vi "Create filename.vi"(9 "Number":i32, 10 "Parameters":T1={"Time"=0.0, "Pixels X"=1, "Pixels Y"=1, "Max galvo"=0.0, "Min galvo"=0.0} {"Pixels Y" min=1; "Pixels X" min=1 step=1; "Time" min=1.0}, 11 "Comment":string) -> (3 "filename":string)   [LabVIEW 2021]
uses:
  Parameters.ctl
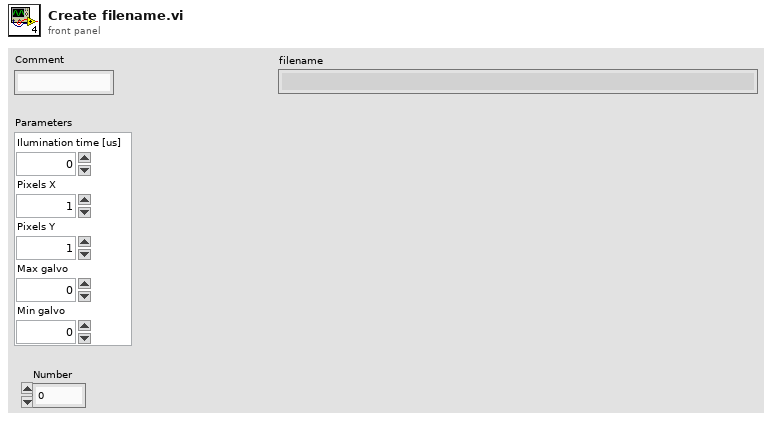
[diagram p1: front panel]
types:
  T1 = typedef "Parameters.ctl" = cluster{"Time":dbl, "Pixels X":i32, "Pixels Y":i32, "Max galvo":dbl, "Min galvo":dbl}
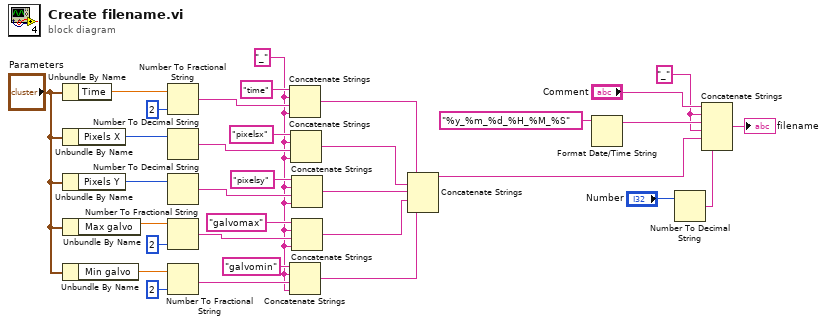
[diagram p0: block diagram]
diagram:
  w9 = "_"
  w31 = "_"
  n1 = Unbundle By Name("Parameters") -> ("Time"=w26:dbl)
  n2 = Unbundle By Name("Parameters") -> ("Pixels X"=w24:i32)
  n3 = Unbundle By Name("Parameters") -> ("Pixels Y"=w23:i32)
  n4 = Unbundle By Name("Parameters") -> ("Max galvo"=w22:dbl)
  n5 = Unbundle By Name("Parameters") -> ("Min galvo"=w25:dbl)
  n6 = Number To Fractional String(number=w26, precision (6)=i16 2) -> (F-format string=w18:string)  [unwired: 2 in]
  n7 = Number To Decimal String(number=w24) -> (decimal integer string=w16:string)  [unwired: 1 in]
  n8 = Number To Decimal String(number=w23) -> (decimal integer string=w14:string)  [unwired: 1 in]
  n9 = Number To Fractional String(number=w22, precision (6)=i16 2) -> (F-format string=w12:string)  [unwired: 2 in]
  n10 = Number To Fractional String(number=w25, precision (6)=i16 2) -> (F-format string=w10:string)  [unwired: 2 in]
  n11 = Concatenate Strings("time" ("string"), w9, w18, w9) -> (w8:string)
  n12 = Concatenate Strings("galvomin" ("string"), w9, w10, w9) -> (w7:string)
  n13 = Concatenate Strings("pixelsx" ("string"), w9, w16, w9) -> (w5:string)
  n14 = Concatenate Strings("pixelsy" ("string"), w9, w14, w9) -> (w4:string)
  n15 = Concatenate Strings("galvomax" ("string"), w9, w12, w9) -> (w6:string)
  n16 = Concatenate Strings(w8, w5, w4, w6, w7) -> (w21:string)
  n17 = Format Date/Time String(time format string (%c)="%y_%m_%d_%H_%M_%S") -> (date/time string=w32:string)  [unwired: 2 in]
  n18 = Number To Decimal String(number="Number") -> (decimal integer string=w20:string)  [unwired: 1 in]
  n19 = Concatenate Strings("Comment", w31, w32, w31, w21, w20) -> (→"filename":string)
